vi "GetText.vi"(8 "error in":errorcluster, 11 "Modbus Slave editor node in":refnum<class "Modbus Module editor node.lvclass">) -> (0 "error out":errorcluster, 1 "additional text":string, 2 "text":string, 3 "Modbus Slave editor node out":refnum<class "Modbus Module editor node.lvclass">, 4 "glyph":string)   [LabVIEW 2015, in "Modbus Module editor node.lvclass"]
doc: "Return the name which the module displays and the glyph is uses within the DCAF tree.\n\nPlatypus Framework 1.0.1.65\nNI Systems Engineering - National Instruments"
uses:
  Modbus Module editor node.lvclass
  <vilib>/NI/DCAF/Tag Editor Core/Configuration Editor/Classes/Module editor node/Read display name.vi
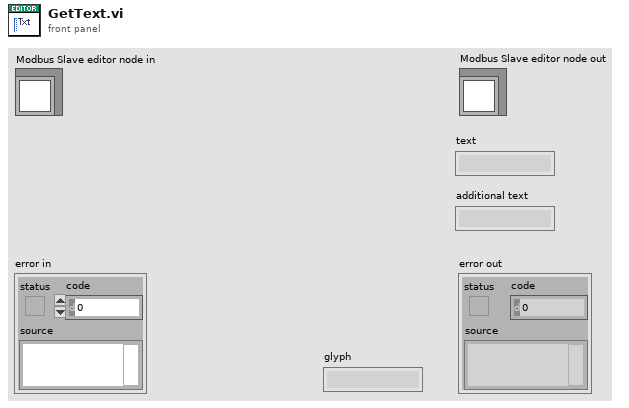
[diagram p1: front panel]
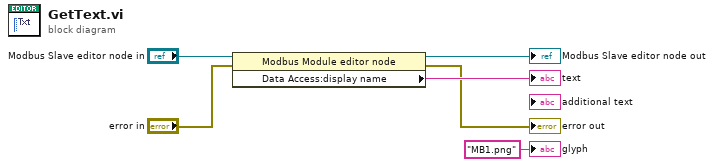
[diagram p0: block diagram]
diagram:
  n1 = property class="Modbus Module editor node"(reference="Modbus Slave editor node in", error in="error in") -> (reference out=→"Modbus Slave editor node out":refnum<class "Modbus Module editor node.lvclass">, error out=→"error out":errorcluster, "Data Access:display name"=→"text":string)
  "glyph" <- "MB1.png" ("glyph")
